vi "Add-table.vi"(7 "F-UP/T-Down":bool, 10 "Indix":i32=3, 11 "数组":string[][](array[string])=[["1", "3"], ["2", "4"], ["新建表1", ""]]) -> (2 "New-table":string, 3 "输出数组":string[][](array[string]))   [LabVIEW 2025]
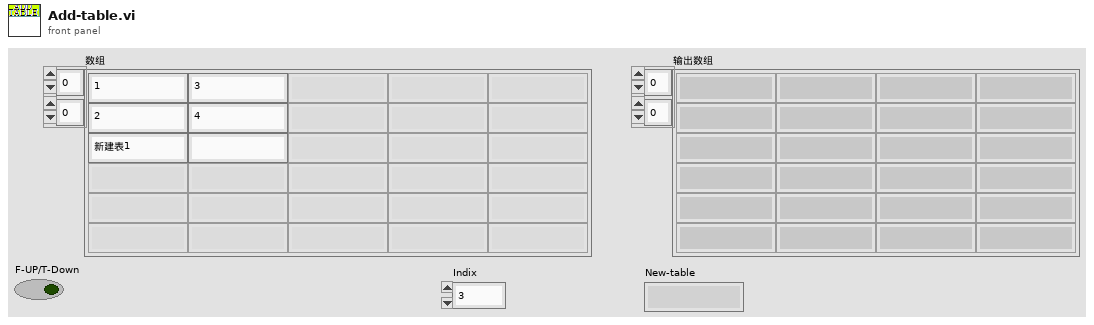
[diagram p1: front panel]
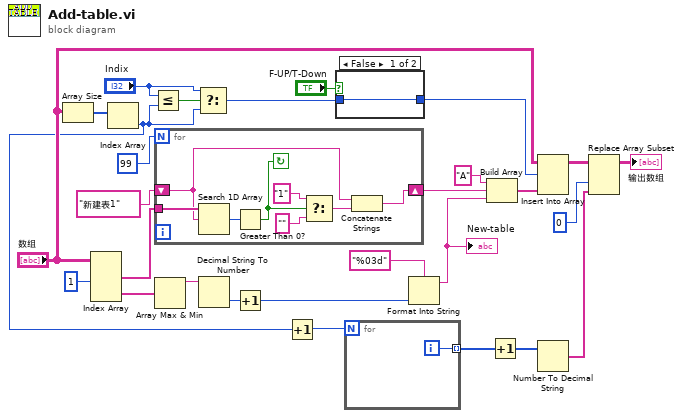
[diagram p0: block diagram]
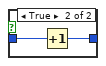
[diagram p2: hidden frame]
diagram:
  n1 = Array Size(array="数组") -> (size(s)=w28:i32[])
  n2 = Index Array(array="数组", index (col) #1=1 ("禁用的索引 (列)")) -> (element #1=w24:string[], element #2=w17:string[])  [unwired: 3 in]
  n3 = Index Array(array=w28) -> (element=w6:i32)  [unwired: 1 in]
  n4 = Less Or Equal?(x="Indix", y=w6) -> (x <= y?=w27:bool)
  n5 = for {
    N: 99 -> [_]
    tunnel: w24 -> [w36]
    shift-right: [w33] -> w21
    shift-left: "新建表1" -> [w34]
    stop <- w32 continue-if-true
    n6 = Search 1D Array(1D array=w36, element=w34) -> (index of element=w35:i32)  [unwired: 1 in]
    n7 = Greater Than 0?(x=w35) -> (x > 0?=w32:bool)
    n8 = Select(t="1" ("字符串"), s=w32, f="") -> (s? t:f=w29:string)
    n9 = Concatenate Strings(w34, w29) -> (w33:string)
  }
  n10 = Array Max & Min(array=w17) -> (max value=w16:string)  [unwired: 3 out]
  n11 = Select(t="Indix", s=w27, f=w6) -> (s? t:f=w18:i32)
  n12 = Decimal String To Number(string=w16) -> (number=w15:i32)  [unwired: 2 in, 1 out]
  n13 = Increment(x=w15) -> (x+1=w14:i32)
  n14 = Increment(x=w6) -> (x+1=w7:i32)
  n15 = case shown="False" "F-UP/T-Down" {
    tunnel: w18 -> [w37 w39]
    tunnel: [w37 w38] -> w2
    frame False {
    }
    frame True {
      n16 = Increment(x=w39) -> (x+1=w38:i32)
    }
  }
  n17 = for {
    N: w7 -> [_]
    tunnel: [w40] -> w5 mode=indexing
    i -> [w40]
  }
  n18 = Format Into String(format string="%03d" ("格式字符串"), w14) -> (resulting string=w12:string)  [unwired: 2 in, 1 out]
  "New-table" <- w12
  n19 = Build Array("A" ("元素"), w21, w12) -> (w20:string[])
  n20 = Increment(x=w5) -> (x+1=w3:i32[])
  n21 = Insert Into Array(array="数组", index (row)=w2, new element=w20) -> (w11:string[][])  [unwired: 1 in]
  n22 = Number To Decimal String(number=w3) -> (decimal integer string=w4:string[])  [unwired: 1 in]
  n23 = Replace Array Subset(array=w11, new element=w4, index (col)=0 ("索引 (行)")) -> (→"输出数组":string[][])  [unwired: 1 in]
